vi "Ecrire config compteurs.vi"(2 "error in (no error)":errorcluster caption="entrée d'erreur (pas d'erreur)", 3 "refnum":T1) -> (0 "error out":errorcluster caption="sortie d'erreur", 1 "refnum out":T1 caption="refnum en sortie")   [LabVIEW 2022 SP3]
uses:
  <vilib>/Utility/config.llb/Config Data RefNum.ctl
  Variables globales/Variable globale compteurs.vi
  <vilib>/Utility/config.llb/Write Key (String).vi
  <vilib>/Utility/config.llb/Write Key (Boolean).vi
  <vilib>/Utility/config.llb/Write Key (Double).vi
  <vilib>/Utility/config.llb/Write Key (U32).vi
  <vilib>/Utility/config.llb/NI_LVConfig.lvlib
panel:
  # "écriture fichier config compteurs"
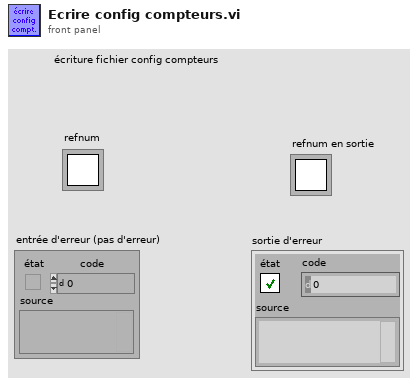
[diagram p1: front panel]
types:
  T1 = typedef "NI_LVConfig.lvlib/Config Data RefNum.ctl" = refnum<k1>
  T2 = cluster{"Nom tache compteurs":refnum<k21>, "Noms des compteurs":string[], "Selection":bool[], "Init compteurs":dbl[], "Noms compteurs selectionnes":string[]}
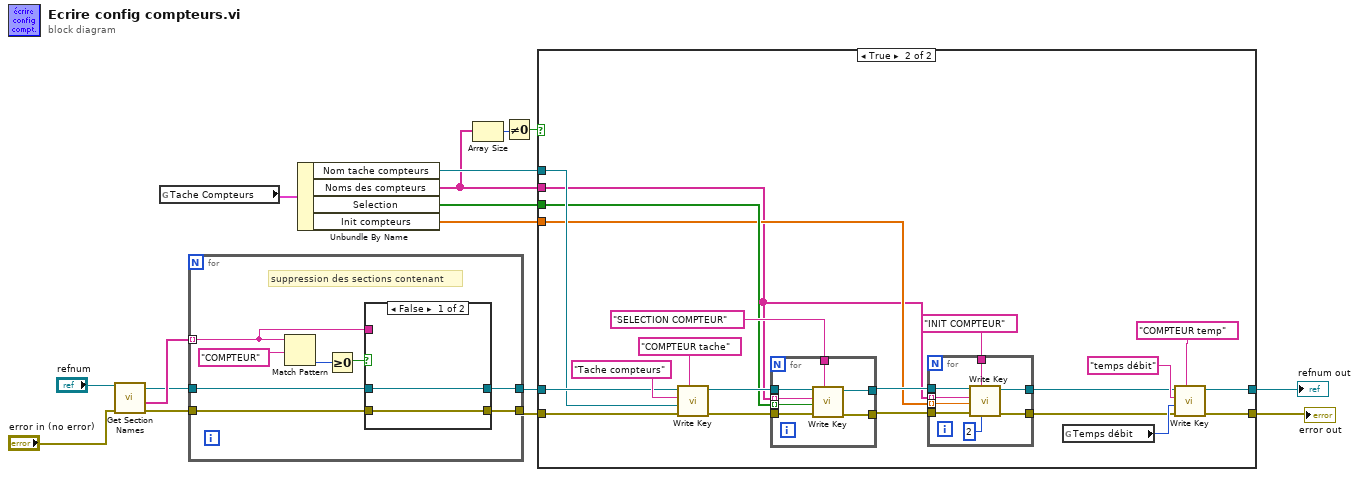
[diagram p0: block diagram]
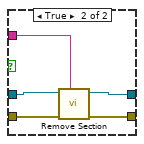
[diagram p3: hidden frame]
diagram:
  n1 = call <vilib>:"Get Section Names.vi"("error in (no error)"="error in (no error)", "refnum"="refnum") -> ("error out"=w15:errorcluster, "section names"=w16:string[], "refnum out"=w14:T1)  [unwired: 7 in]
  n2 = global read "Variable globale compteurs.vi" "Tache Compteurs"() -> (w11:T2)
  n3 = for {
    tunnel: w16 -> [w21] mode=indexing
    tunnel: w15 -> [w19]
    tunnel: [w17] -> w9
    tunnel: w14 -> [w20]
    tunnel: [w18] -> w10
    # "suppression des sections contenant"
    n4 = Match Pattern(string=w21, regular expression="COMPTEUR" ("expression régulière")) -> (offset past match=w23:i32)  [unwired: 1 in, 3 out]
    n5 = Greater Or Equal To 0?(x=w23) -> (x >= 0?=w22:bool)
    n6 = case shown="False" w22 {
      tunnel: w21 -> [_ w31]
      tunnel: w20 -> [w26 w29]
      tunnel: w19 -> [w25 w30]
      tunnel: [w26 w28] -> w18
      tunnel: [w25 w27] -> w17
      frame False {
      }
      frame True {
        n7 = call <vilib>:"Remove Section.vi"("section"=w31, "error in (no error)"=w30, "refnum"=w29) -> ("error out"=w27:errorcluster, "refnum out"=w28:T1)  [unwired: 6 in, 1 out]
      }
    }
  }
  n8 = Unbundle By Name(w11) -> ("Nom tache compteurs"=w8:refnum<k21>, "Noms des compteurs"=w3:string[], "Selection"=w7:bool[], "Init compteurs"=w6:dbl[])
  n9 = Array Size(array=w3) -> (size(s)=w2:i32)
  n10 = Not Equal To 0?(x=w2) -> (x != 0?=w1:bool)
  n11 = case shown="True" w1 {
    tunnel: w10 -> [w33 w52]
    tunnel: w9 -> [w32 w51]
    tunnel: w8 -> [_ w50]
    tunnel: w7 -> [_ w46]
    tunnel: w6 -> [_ w43]
    tunnel: [w33 w36] -> w5
    tunnel: [w32 w37] -> w4
    tunnel: w3 -> [_ w41]
    frame False {
    }
    frame True {
      n12 = call-poly <vilib>:"Write Key.vi"("section"="COMPTEUR tache", "error in (no error)"=w51, "value"=w50, "key"="Tache compteurs", "refnum"=w52) -> ("error out"=w47:errorcluster, "refnum out"=w49:T1)  [unwired: 4 in, 1 out]
      n13 = for {
        tunnel: w41 -> [w69] mode=indexing
        tunnel: w49 -> [w68]
        tunnel: "SELECTION COMPTEUR" ("section") -> [w67]
        tunnel: w47 -> [w66]
        tunnel: w46 -> [w65] mode=indexing
        tunnel: [w64] -> w45
        tunnel: [w63] -> w44
        n14 = call-poly <vilib>:"Write Key.vi"("section"=w67, "error in (no error)"=w66, "value"=w65, "key"=w69, "refnum"=w68) -> ("error out"=w63:errorcluster, "refnum out"=w64:T1)  [unwired: 4 in, 1 out]
      }
      n15 = for {
        tunnel: w41 -> [w62] mode=indexing
        tunnel: w45 -> [w61]
        tunnel: "INIT COMPTEUR" ("section") -> [w60]
        tunnel: w44 -> [w59]
        tunnel: w43 -> [w58] mode=indexing
        tunnel: [w57] -> w35
        tunnel: [w56] -> w34
        n16 = call-poly <vilib>:"Write Key.vi"("precision (6)"=i16 2, "section"=w60, "error in (no error)"=w59, "value"=w58, "key"=w62, "refnum"=w61) -> ("error out"=w56:errorcluster, "refnum out"=w57:T1)  [unwired: 3 in, 1 out]
      }
      n17 = global read "Variable globale compteurs.vi" "Temps débit"() -> (w38:u16)
      n18 = call-poly <vilib>:"Write Key.vi"("section"="COMPTEUR temp", "error in (no error)"=w34, "value"=w38, "key"="temps débit", "refnum"=w35) -> ("error out"=w37:errorcluster, "refnum out"=w36:T1)  [unwired: 4 in, 1 out]
    }
  }
  "refnum out" <- w5
  "error out" <- w4
